vi "VM - Initializing.vi"(8 "error in":errorcluster) -> (0 "error out":errorcluster, 1 "err code":T1 items=["No error", "Invalid variable type", "Variable not found", "Variable already exists", "Invalid context handle", "Input error", "Invalid data format", "No history attached", "History already attached", "Invalid history parameters", "Wrong variable name", "Wrong alias name", "Non-unique alias", "Alias not found", "No alias associated", "Alias already associated", "Wrong context name", "Non-unique context name", "Context name not found", "Invalid parameter", "Generic error", "Memory Full", "Unrecognized LV error", "Unknown error code"])   [LabVIEW 2021]
doc: "This VI initializes VarMan. When this VI completes, all local variable contexts are closed and all variables are destroyed. Refer to the VI help for more details.\n\n::: CalcExpress Toolkit :::\nCopyright (c) 2000-2026 Konstantin Shifershteyn. All rights reserved."
uses:
  cetypes.llb/VarMan Error Code.ctl
  cersrc/celveng32.dll
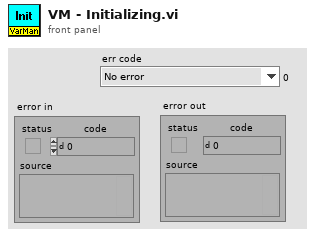
[diagram p1: front panel]
types:
  T1 = typedef "VarMan Error Code.ctl" = u16
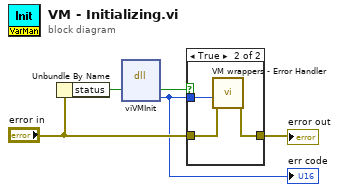
[diagram p0: block diagram]
diagram:
  n1 = Unbundle By Name("error in") -> ("status"=w3:bool)
  n2 = dll-call lib="C:/LV Projects/CalcExpress 40 LV2021/vi.lib/addons/CalcExpress/cersrc/celveng*.dll" fn="viVMInit"("errf"=w3) -> ("errf"=w2:bool, "err code"=w1:T1)  [unwired: 5 in, 2 out]
  "err code" <- w1
  n3 = case shown="True" w2 {
    tunnel: [w6 w9] -> w5
    tunnel: "error in" -> [w6 w8]
    tunnel: w1 -> [_ w7]
    frame False {
    }
    frame True {
      n4 = call "VM wrappers - Error Handler.vi"("error before"=w8, "VarMan error"=w7) -> ("error out"=w9:errorcluster)  [unwired: 8 in, 1 out]
    }
  }
  "error out" <- w5
